vi "Run Test (Scalar Path).vi"(4 "timeout (2000 ms)":i32=2000, 5 "Test Report":refnum<class "Test Report.lvclass">, 6 "Verbose":bool, 7 "Report Path":path, 8 "error in":errorcluster, 9 "Inspect Recursively (T)":bool=TRUE, 10 "Test Path":path, 11 "Interactive (T)":bool=TRUE) -> (0 "error out":errorcluster, 3 "Test Results":refnum<class "Test Result.lvclass">)   [LabVIEW 2020, in "Caraya.lvlib"]
doc: "\"Run Tests\" from a path (folder or VI):\n- Dynamically discovers Caraya unit tests and runs them based on VI path or folder\n- Outputs results in a UI ans/or Test Report (J-Unit or text)\n\n(Not compatible with RT targets or RunTime Engine)"
uses:
  Caraya.lvlib
  classes/Test Report/Test Report.lvclass
  classes/Test Result/Test Result.lvclass
  classes/Test Runner.Folder/Test Runner.Folder.lvclass
  C:/projects/caraya/src/classes/Test Runner/Test Runner.lvclass
  classes/Test Runner.Class/Test Runner.Class.lvclass
  classes/Test Runner.Project/Test Runner.Project.lvclass
  classes/Test Runner.Library/Test Runner.Library.lvclass
  <userlib>/_OpenG.lib/file/file.llb/Valid Path - Traditional__ogtk.vi
  <userlib>/_OpenG.lib/file/file.llb/File Exists - Scalar__ogtk.vi
  <userlib>/_OpenG.lib/file/file.llb/Strip Path Extension - Path__ogtk.vi
  classes/Test Runner/Test Runner.lvclass
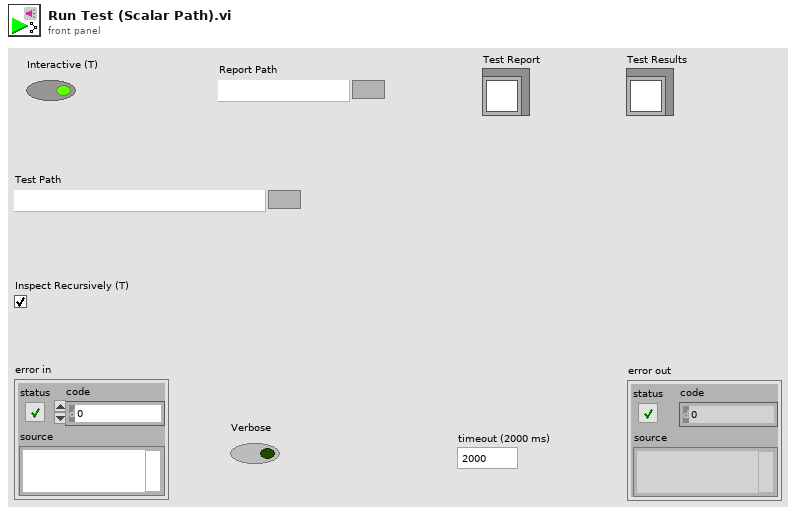
[diagram p1: front panel]
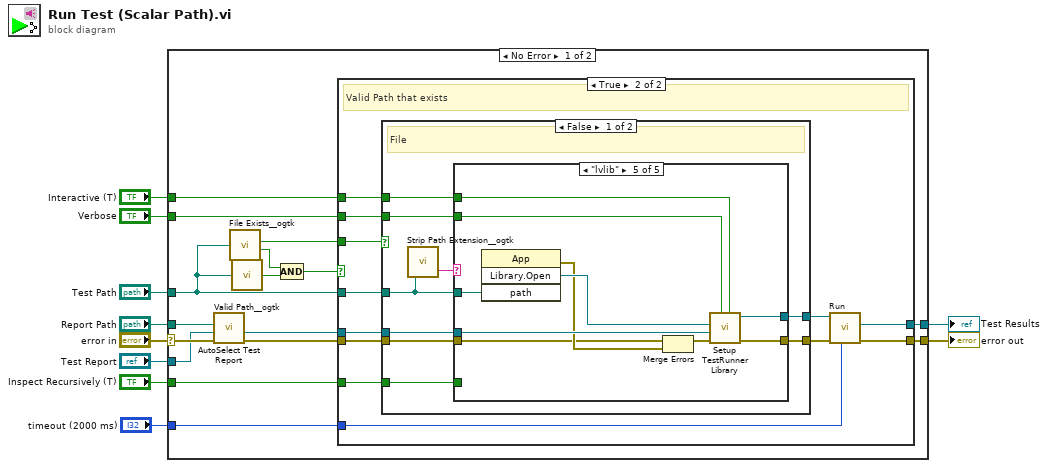
[diagram p0: block diagram]
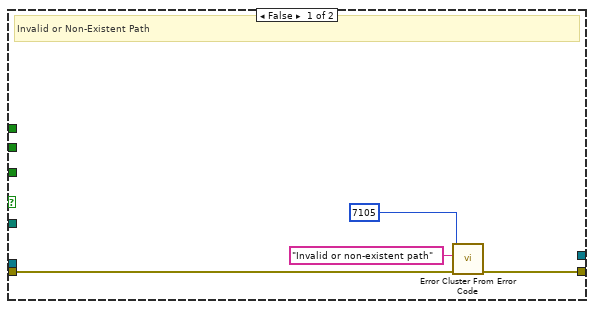
[diagram p2: hidden frame]
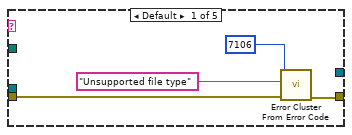
[diagram p3: hidden frame]
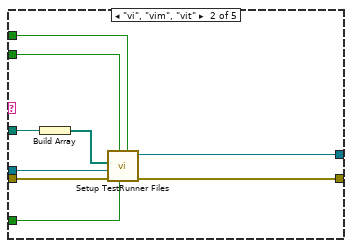
[diagram p4: hidden frame]
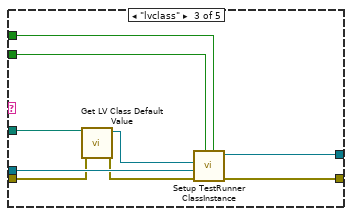
[diagram p5: hidden frame]
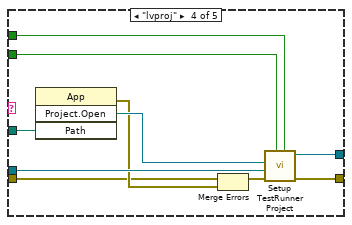
[diagram p6: hidden frame]
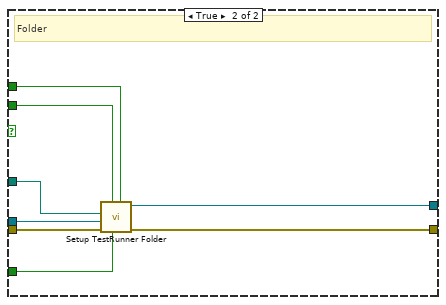
[diagram p7: hidden frame]
diagram:
  n1 = case shown="No Error" "error in" {
    selector: "error in" -> [w23 w102]
    tunnel: [w26 w102] -> w10
    tunnel: "Verbose" -> [w25 _]
    tunnel: "Interactive (T)" -> [w24 _]
    tunnel: "Test Report" -> [w20 _]
    tunnel: "Test Path" -> [w16 _]
    tunnel: "Report Path" -> [w22 _]
    tunnel: "Inspect Recursively (T)" -> [w17 _]
    tunnel: "timeout (2000 ms)" -> [w12 _]
    tunnel: [w11 _] -> w1
    frame No Error {
      n2 = call "AutoSelect Test Report.vi"("error in (no error)"=w23, "Test Report in"=w20, "Report Path"=w22) -> ("error out"=w21:errorcluster, "Test Report out"=w19:refnum<class "Test Report.lvclass">)  [unwired: 7 in]
      n3 = call-poly <userlib>:"File Exists__ogtk.vi"("file path"=w16) -> ("is directory"=w13:bool, "exists"=w18:bool)  [unwired: 6 in]
      n4 = call-poly <userlib>:"Valid Path__ogtk.vi"("path"=w16) -> ("valid"=w15:bool)
      n5 = Compound Arithmetic op=AND(w18, w15) -> (w14:bool)
      n6 = case shown="True" w14 {
        tunnel: [w29 w42] -> w26
        tunnel: w25 -> [_ w40]
        tunnel: w24 -> [_ w39]
        tunnel: w21 -> [w30 w37]
        tunnel: w19 -> [_ w36]
        tunnel: w17 -> [_ w35]
        tunnel: w16 -> [_ w34]
        tunnel: w13 -> [_ w33]
        tunnel: w12 -> [_ w32]
        tunnel: [_ w31] -> w11
        frame False {
          # "Invalid or Non-Existent Path"
          n7 = call <vilib>:"Error Cluster From Error Code.vi"("error in (no error)"=w30, "error message (\"\")"="Invalid or non-existent path" ("error message (\"\")"), "error code (0)"=7105 ("code")) -> ("error out"=w29:errorcluster)  [unwired: 6 in]
        }
        frame True {
          # "Valid Path that exists"
          n8 = case shown="False" w33 {
            tunnel: [w50 w101] -> w41
            tunnel: w40 -> [w47 w100]
            tunnel: w39 -> [w48 w99]
            tunnel: [w49 w98] -> w38
            tunnel: w37 -> [w51 w97]
            tunnel: w36 -> [w46 w96]
            tunnel: w34 -> [w44 w95]
            tunnel: w35 -> [w45 w94]
            frame False {
              # "File"
              n9 = call-poly <userlib>:"Strip Path Extension__ogtk.vi"("path"=w44) -> ("extension"=w43:string)  [unwired: 1 out]
              n10 = case shown="\"lvlib\"" w43 {
                tunnel: w51 -> [w53 w64 w67 w75 w85]
                tunnel: [w52 w63 w73 w82 w92] -> w50
                tunnel: [_ w62 w72 w83 w93] -> w49
                tunnel: w48 -> [_ w61 w71 w79 w89]
                tunnel: w47 -> [_ w60 w70 w80 w90]
                tunnel: w46 -> [_ w59 w69 w81 w91]
                tunnel: w45 -> [_ w58 _ _ _]
                tunnel: w44 -> [_ w56 w68 w78 w88]
                frame Default {
                  n11 = call <vilib>:"Error Cluster From Error Code.vi"("error in (no error)"=w53, "error message (\"\")"="Unsupported file type" ("error message (\"\")"), "error code (0)"=7106 ("code")) -> ("error out"=w52:errorcluster)  [unwired: 6 in]
                }
                frame "vi", "vim", "vit" {
                  n12 = Build Array(w56) -> (w57:path[])
                  n13 = call "Setup TestRunner Files.vi"("Interactive (T)"=w61, "Inspect Recursively (T)"=w58, "Verbose (F)"=w60, "error in (no error)"=w64, "Test Report"=w59, "Paths"=w57) -> ("error out"=w63:errorcluster, "Test Runner.Folder out"=w62:refnum<class "Test Runner.Folder.lvclass">)  [unwired: 4 in]
                }
                frame "lvclass" {
                  n14 = call <vilib>:"Get LV Class Default Value.vi"("error in (no error)"=w67, "class path"=w68) -> ("error out"=w66:errorcluster, "object"=w65:refnum<class>)  [unwired: 8 in]
                  n15 = call "Setup TestRunner ClassInstance.vi"("Interactive (T)"=w71, "Verbose (F)"=w70, "error in (no error)"=w66, "Test Report"=w69, "Instance"=w65) -> ("error out"=w73:errorcluster, "Test Runner.Class out"=w72:refnum<class "Test Runner.Class.lvclass">)  [unwired: 5 in]
                }
                frame "lvproj" {
                  n16 = invoke class="App" method="Project.Open"("Path"=w78) -> (error out=w76:errorcluster, "Project:Open"=w77:refnum<vi>)  [unwired: 3 in, 2 out]
                  n17 = Merge Errors(w75, w76) -> (w74:errorcluster)
                  n18 = call "Setup TestRunner Project.vi"("Interactive (T)"=w79, "Verbose (F)"=w80, "error in (no error)"=w74, "Test Report"=w81, "Project Refnum"=w77) -> ("error out"=w82:errorcluster, "Test Runner.Project out"=w83:refnum<class "Test Runner.Project.lvclass">)  [unwired: 5 in]
                }
                frame "lvlib" {
                  n19 = invoke class="App" method="Library.Open"("path"=w88) -> (error out=w86:errorcluster, "Open Library"=w87:refnum<vi>)  [unwired: 3 in, 2 out]
                  n20 = Merge Errors(w85, w86) -> (w84:errorcluster)
                  n21 = call "Setup TestRunner Library.vi"("Interactive (T)"=w89, "Verbose (F)"=w90, "error in (no error)"=w84, "Test Report"=w91, "Library Refnum"=w87) -> ("error out"=w92:errorcluster, "Test Runner.Library out"=w93:refnum<class "Test Runner.Library.lvclass">)  [unwired: 5 in]
                }
              }
            }
            frame True {
              # "Folder"
              n22 = call "Setup TestRunner Folder.vi"("Interactive (T)"=w99, "Inspect Recursively (T)"=w94, "Verbose (F)"=w100, "error in (no error)"=w97, "Test Report"=w96, "Directory to search"=w95) -> ("error out"=w101:errorcluster, "Test Runner.Folder out"=w98:refnum<class "Test Runner.Folder.lvclass">)  [unwired: 4 in]
            }
          }
          n23 = call "Run.vi"("timeout"=w32, "error in (no error)"=w41, "Test Runner in"=w38) -> ("error out"=w42:errorcluster, "Test Suite Results"=w31:refnum<class "Test Result.lvclass">)  [unwired: 6 in, 1 out]
        }
      }
    }
    frame Error {
    }
  }
  "error out" <- w10
  "Test Results" <- w1
